vi "[ce] Get Win File Version.vi"(8 "error in":errorcluster, 11 "File path":path) -> (0 "error out":errorcluster, 2 "File Info":T1, 3 "dup File path":path)   [LabVIEW 2021]
doc: "::: CalcExpress Toolkit :::\nCopyright (c) 2000-2026 Konstantin Shifershteyn. All rights reserved."
uses:
  version.dll
  kernel32.dll
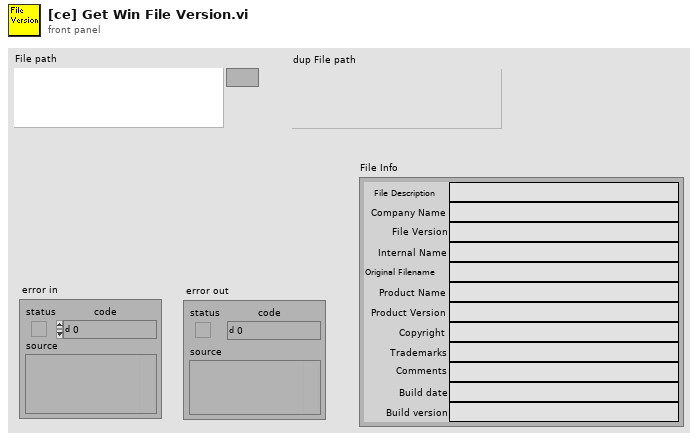
[diagram p1: front panel]
types:
  T1 = cluster{"File Description":string, "Company Name":string, "File Version":string, "Internal Name":string, "Original Filename":string, "Product Name":string, "Product Version":string, "Copyright":string, "Trademarks":string, "Comments":string, "Build date":string, "Build version":string}
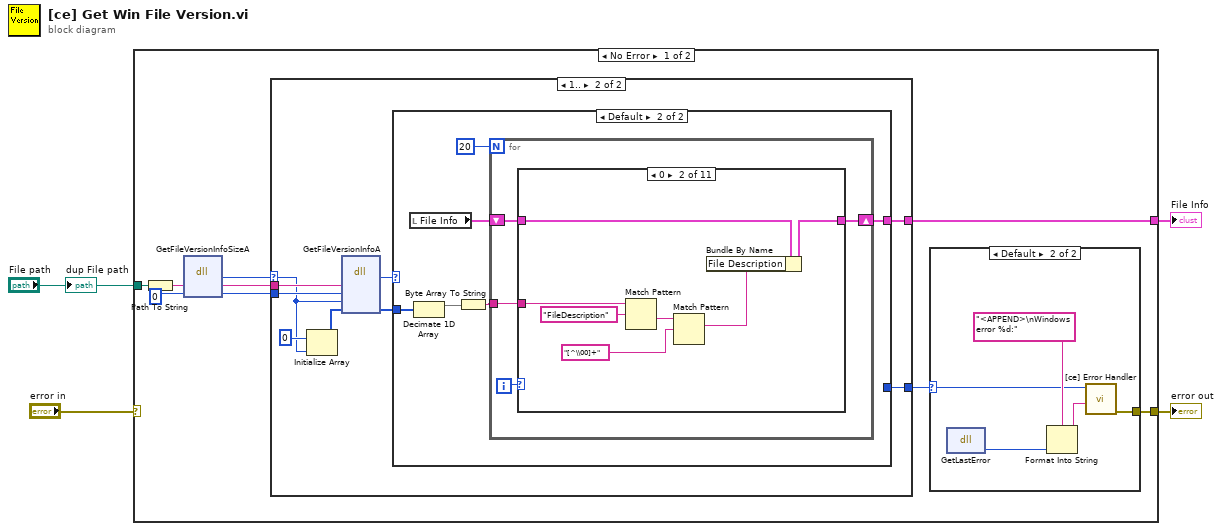
[diagram p0: block diagram]
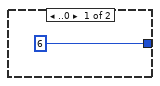
[diagram p3: hidden frame]
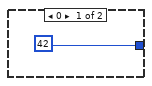
[diagram p4: hidden frame]
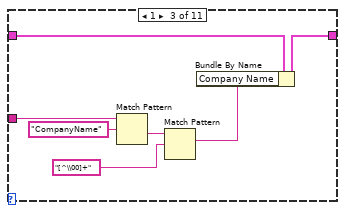
[diagram p6: hidden frame]
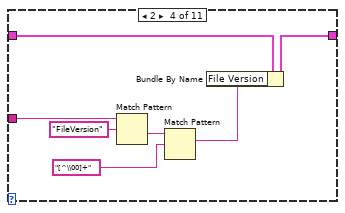
[diagram p7: hidden frame]
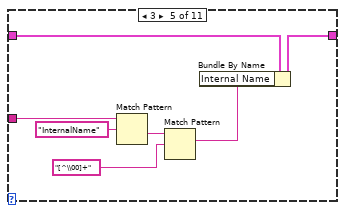
[diagram p8: hidden frame]
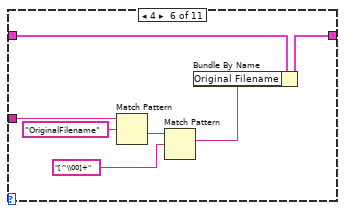
[diagram p9: hidden frame]
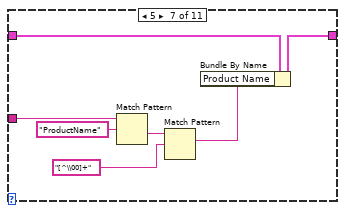
[diagram p10: hidden frame]
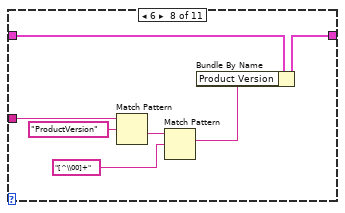
[diagram p11: hidden frame]
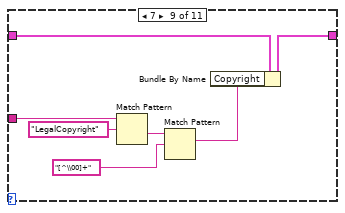
[diagram p12: hidden frame]
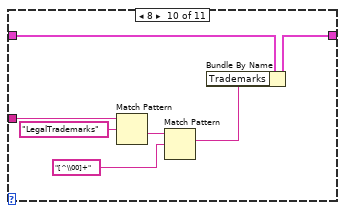
[diagram p13: hidden frame]
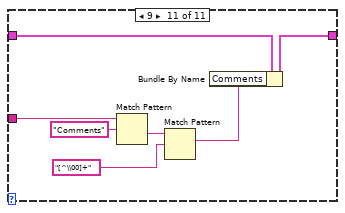
[diagram p14: hidden frame]
diagram:
  n1 = case shown="No Error" "error in" {
    selector: "error in" -> [_ w111]
    tunnel: [w8 _] -> w4
    tunnel: "File path" -> [w7 _]
    tunnel: [w6 w111] -> w1
    frame No Error {
      n2 = Path To String(path=w7) -> (string=w12:string)
      n3 = dll-call lib="version.dll" fn="GetFileVersionInfoSizeA" label="version.dll:\nGetFileVersionInfoSizeA"("FilePath"=w12, "null"=0) -> ("size"=w11:i32, "FilePath"=w10:string, "null"=w9:i32)  [unwired: 3 in, 2 out]
      n4 = case shown="1.." w11 {
        selector: w11 -> [_ w25]
        tunnel: w10 -> [_ w28]
        tunnel: w9 -> [_ w27]
        tunnel: [_ w22] -> w8
        tunnel: [6 ("error code") w20] -> w5
        frame ..0 {
        }
        frame 1.. {
          n5 = Initialize Array(u8 0, w25) -> (w24:u8[])
          n6 = dll-call lib="version.dll" fn="GetFileVersionInfoA" label="version.dll:\nGetFileVersionInfoA"("FilePath"=w28, "null"=w27, "size"=w25, "Buffer"=w24) -> ("return type"=w21:i32, "Buffer"=w23:u8[])  [unwired: 6 in, 2 out]
          n7 = case shown="Default" w21 {
            tunnel: w23 -> [_ w30]
            tunnel: [_ w33] -> w22
            tunnel: [42 _] -> w20
            frame 0 {
            }
            frame Default {
              n8 = local read "File Info"() -> (w34:T1)
              n9 = Decimate 1D Array(w30) -> (w31:u8[])  [unwired: 1 out]
              n10 = Byte Array To String(unsigned byte array=w31) -> (string=w32:string)
              n11 = for {
                N: 20 -> [_]
                tunnel: w32 -> [w39]
                shift-right: [w36] -> w33
                shift-left: w34 -> [w37]
                i -> [w38]
                n12 = case shown="0" w38 {
                  tunnel: w39 -> [_ w45 w52 w59 w66 w73 w80 w87 w94 w101 w108]
                  tunnel: w37 -> [w40 w43 w50 w57 w64 w71 w78 w85 w92 w99 w106]
                  tunnel: [w40 w42 w49 w56 w63 w70 w77 w84 w91 w98 w105] -> w36
                  frame Default {
                  }
                  frame 0 {
                    n13 = Match Pattern(string=w45, regular expression="FileDescription" ("search string/char (-)")) -> (after substring=w44:string)  [unwired: 1 in, 3 out]
                    n14 = Match Pattern(string=w44, regular expression="[^\\00]+") -> (match substring=w41:string)  [unwired: 1 in, 3 out]
                    n15 = Bundle By Name(cluster=w43, "File Description"=w41) -> (w42:T1)
                  }
                  frame 1 {
                    n16 = Match Pattern(string=w52, regular expression="CompanyName" ("search string/char (-)")) -> (after substring=w51:string)  [unwired: 1 in, 3 out]
                    n17 = Match Pattern(string=w51, regular expression="[^\\00]+") -> (match substring=w48:string)  [unwired: 1 in, 3 out]
                    n18 = Bundle By Name(cluster=w50, "Company Name"=w48) -> (w49:T1)
                  }
                  frame 2 {
                    n19 = Match Pattern(string=w59, regular expression="FileVersion" ("search string/char (-)")) -> (after substring=w58:string)  [unwired: 1 in, 3 out]
                    n20 = Match Pattern(string=w58, regular expression="[^\\00]+") -> (match substring=w55:string)  [unwired: 1 in, 3 out]
                    n21 = Bundle By Name(cluster=w57, "File Version"=w55) -> (w56:T1)
                  }
                  frame 3 {
                    n22 = Match Pattern(string=w66, regular expression="InternalName" ("search string/char (-)")) -> (after substring=w65:string)  [unwired: 1 in, 3 out]
                    n23 = Match Pattern(string=w65, regular expression="[^\\00]+") -> (match substring=w62:string)  [unwired: 1 in, 3 out]
                    n24 = Bundle By Name(cluster=w64, "Internal Name"=w62) -> (w63:T1)
                  }
                  frame 4 {
                    n25 = Match Pattern(string=w73, regular expression="OriginalFilename" ("search string/char (-)")) -> (after substring=w72:string)  [unwired: 1 in, 3 out]
                    n26 = Match Pattern(string=w72, regular expression="[^\\00]+") -> (match substring=w69:string)  [unwired: 1 in, 3 out]
                    n27 = Bundle By Name(cluster=w71, "Original Filename"=w69) -> (w70:T1)
                  }
                  frame 5 {
                    n28 = Match Pattern(string=w80, regular expression="ProductName" ("search string/char (-)")) -> (after substring=w79:string)  [unwired: 1 in, 3 out]
                    n29 = Match Pattern(string=w79, regular expression="[^\\00]+") -> (match substring=w76:string)  [unwired: 1 in, 3 out]
                    n30 = Bundle By Name(cluster=w78, "Product Name"=w76) -> (w77:T1)
                  }
                  frame 6 {
                    n31 = Match Pattern(string=w87, regular expression="ProductVersion" ("search string/char (-)")) -> (after substring=w86:string)  [unwired: 1 in, 3 out]
                    n32 = Match Pattern(string=w86, regular expression="[^\\00]+") -> (match substring=w83:string)  [unwired: 1 in, 3 out]
                    n33 = Bundle By Name(cluster=w85, "Product Version"=w83) -> (w84:T1)
                  }
                  frame 7 {
                    n34 = Match Pattern(string=w94, regular expression="LegalCopyright" ("search string/char (-)")) -> (after substring=w93:string)  [unwired: 1 in, 3 out]
                    n35 = Match Pattern(string=w93, regular expression="[^\\00]+") -> (match substring=w90:string)  [unwired: 1 in, 3 out]
                    n36 = Bundle By Name(cluster=w92, "Copyright"=w90) -> (w91:T1)
                  }
                  frame 8 {
                    n37 = Match Pattern(string=w101, regular expression="LegalTrademarks" ("search string/char (-)")) -> (after substring=w100:string)  [unwired: 1 in, 3 out]
                    n38 = Match Pattern(string=w100, regular expression="[^\\00]+") -> (match substring=w97:string)  [unwired: 1 in, 3 out]
                    n39 = Bundle By Name(cluster=w99, "Trademarks"=w97) -> (w98:T1)
                  }
                  frame 9 {
                    n40 = Match Pattern(string=w108, regular expression="Comments" ("search string/char (-)")) -> (after substring=w107:string)  [unwired: 1 in, 3 out]
                    n41 = Match Pattern(string=w107, regular expression="[^\\00]+") -> (match substring=w104:string)  [unwired: 1 in, 3 out]
                    n42 = Bundle By Name(cluster=w106, "Comments"=w104) -> (w105:T1)
                  }
                }
              }
            }
          }
        }
      }
      n43 = case shown="Default" w5 {
        selector: w5 -> [_ w16]
        tunnel: [_ w15] -> w6
        frame 0 {
        }
        frame Default {
          n44 = dll-call lib="kernel32.dll" fn="GetLastError" label="kernel32.dll:\nGetLastError"() -> ("return type"=w17:i32)  [unwired: 3 in, 2 out]
          n45 = Format Into String(format string="<APPEND>\nWindows error %d:", w17) -> (resulting string=w14:string)  [unwired: 2 in, 1 out]
          n46 = call "[ce] Error Handler.vi"("error reason"=w14, "error code"=w16) -> ("error out"=w15:errorcluster)  [unwired: 8 in, 1 out]
        }
      }
    }
    frame Error {
    }
  }
  "File Info" <- w4
  "error out" <- w1
  "dup File path" <- "File path"
